vi "Hud_Blit.vi"(0 "Picture":u8[][](array[numeric]), 5 "Sprites":cluster{"Pix":u8[][], "Mask":u8[][]}[](array[cluster]), 7 "State":T1={"Tick"=0, "Phase"=0, "PhaseTicks"=0, "Level"=1, "Room"=0, "X10"=0, "Y10"=0, "VY10"=0, "Mode"=0, "Facing"=0, "Run"=0, "Vert"=0, "StandY"=0, "EntryX10"=0, "EntryY10"=0, "EntryMode"=0, "Lives"=4, "Score"=0, "NextLife"=10000, "KeyR"=0, "KeyB"=0, "KeyY"=0, "Torch"=FALSE, "FloorPhase"=0, "Dead"=FALSE, "LevelStart"=FALSE, "Quit"=FALSE, "Sound"=0, "Seed"=12345, "DemoStep"=0, "Tiles"=[], "World"=[], "Enemies"=[], "Highscores"=[], "Name"=[0, 0, 0], "Cursor"=0}, 11 "error in":errorcluster) -> (4 "Picture out":u8[][](array[numeric]), 15 "error out":errorcluster)   [LabVIEW 2020, in "GH_Render.lvlib"]
doc: "Draws the HUD values into the screen raster (the HUD image itself is already there): lives (at most 7 heads), keys with their number, the torch, level, gold (score) and in the treasure room the seconds left."
uses:
  GH_Render.lvlib
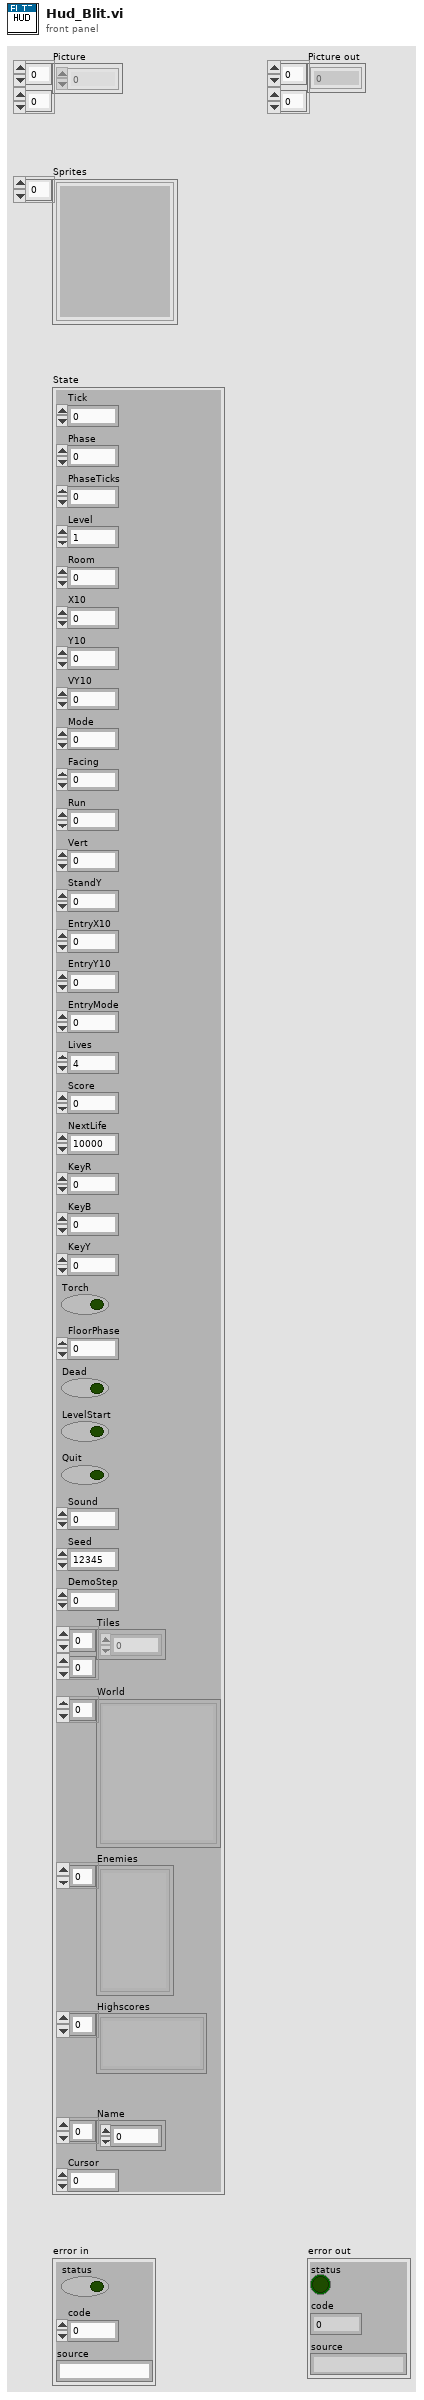
[diagram p1: front panel]
types:
  T1 = cluster{"Tick":u32, "Phase":i32, "PhaseTicks":i32, "Level":i32, "Room":i32, "X10":i32, "Y10":i32, "VY10":i32, "Mode":i32, "Facing":i32, "Run":i32, "Vert":i32, "StandY":i32, "EntryX10":i32, "EntryY10":i32, "EntryMode":i32, "Lives":i32, "Score":i32, "NextLife":i32, "KeyR":i32, "KeyB":i32, "KeyY":i32, "Torch":bool, "FloorPhase":i32, "Dead":bool, "LevelStart":bool, "Quit":bool, "Sound":i32, "Seed":u32, "DemoStep":i32, "Tiles":u8[][], "World":cluster{"ID":string, "Depth":i32, "Column":i32, "Tiles":u8[][]}[], "Enemies":cluster{"Kind":i32, "X10":i32, "Y10":i32, "Dir":i32, "Mode":i32}[], "Highscores":cluster{"Score":i32, "Name":string}[], "Name":i32[], "Cursor":i32}
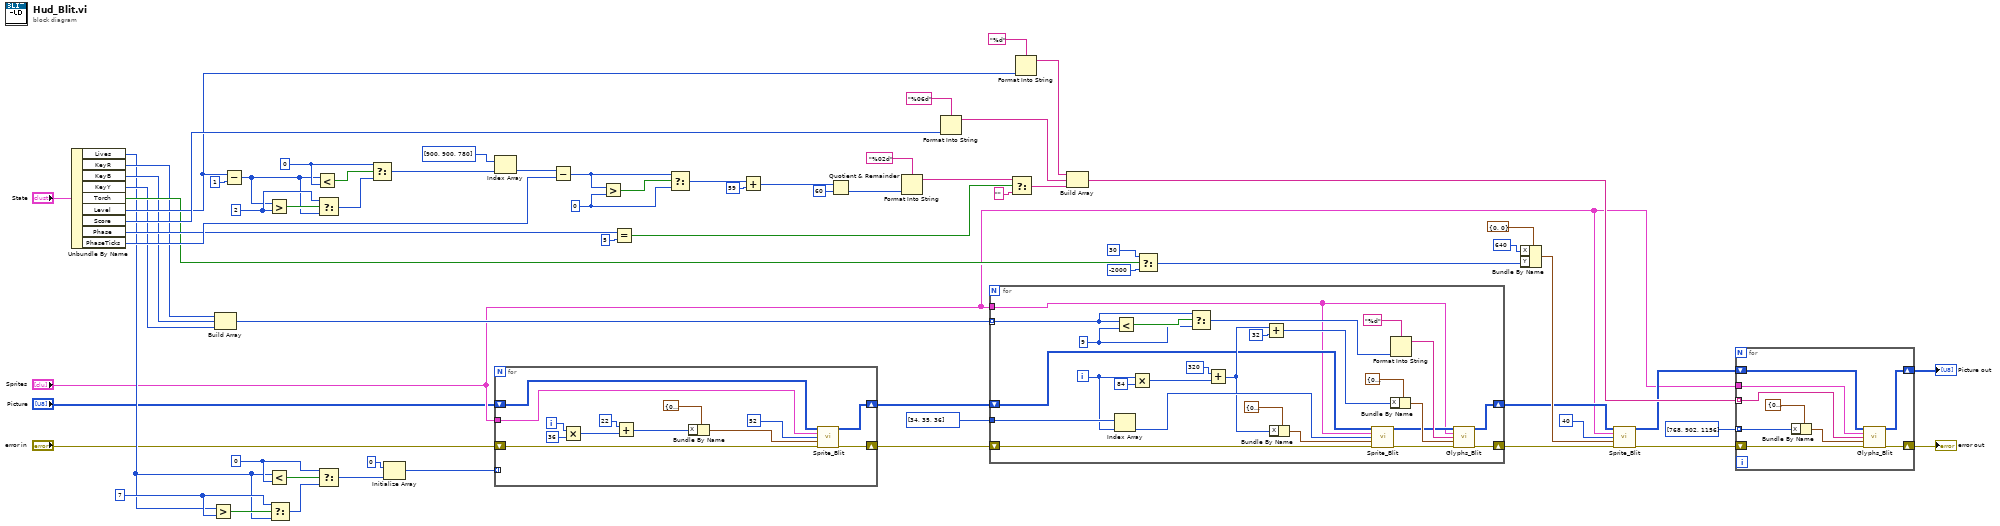
[diagram p0: block diagram]
diagram:
  w48 = 0
  w41 = 2
  w40 = 0
  w15 = 7
  w14 = 0
  n1 = Unbundle By Name("State") -> ("Lives"=w5:i32, "KeyR"=w6:i32, "KeyB"=w7:i32, "KeyY"=w8:i32, "Torch"=w9:bool, "Level"=w10:i32, "Score"=w11:i32, "Phase"=w12:i32, "PhaseTicks"=w13:i32)
  n2 = Greater?(x=w5, y=w15) -> (0:w17:bool)
  n3 = Build Array(w6, w7, w8) -> (w24:i32[])
  n4 = Subtract(x=w10, y=1) -> (x-y=w39:i32)
  n5 = Greater?(x=w39, y=w41) -> (0:w43:bool)
  n6 = Less?(x=w5, y=w14) -> (x < y?=w16:bool)
  n7 = Select(t=w15, s=w17, f=w5) -> (s? t:f=w18:i32)
  n8 = Less?(x=w39, y=w40) -> (x < y?=w42:bool)
  n9 = Select(t=w41, s=w43, f=w39) -> (s? t:f=w44:i32)
  n10 = Select(t=w14, s=w16, f=w18) -> (s? t:f=w19:i32)
  n11 = Select(t=w40, s=w42, f=w44) -> (s? t:f=w45:i32)
  n12 = Initialize Array(0, w19) -> (w21:i32[])
  n13 = Index Array(array=i32[] [900, 900, 780] ("Treasure time"), index=w45) -> (element=w46:i32)
  n14 = for {
    tunnel: "Sprites" -> [w70]
    shift-right: [w72] -> w22
    shift-left: "Picture" -> [w71]
    shift-right: [w74] -> w23
    shift-left: "error in" -> [w73]
    tunnel: w21 -> [_] mode=indexing
    i -> [w69]
    n15 = Multiply(x=w69, y=36) -> (x*y=w79:i32)
    n16 = Add(x=22, y=w79) -> (x+y=w80:i32)
    n17 = Bundle By Name(cluster=cluster{"X":i32, "Y":i32} {"X"=0, "Y"=30}, "X"=w80) -> (w81:cluster{"X":i32, "Y":i32})
    n18 = call "Sprite_Blit.vi"("Picture"=w71, "Sprites"=w70, "Index"=52, "Position"=w81, "error in"=w73) -> ("Picture out"=w72:u8[][], "error out"=w74:errorcluster)  [unwired: 9 in]
  }
  n19 = Subtract(x=w46, y=w13) -> (x-y=w47:i32)
  n20 = Greater?(x=w47, y=w48) -> (0:w49:bool)
  n21 = Equal?(x=w12, y=5) -> (x = y?=w56:bool)
  n22 = Select(t=w47, s=w49, f=w48) -> (s? t:f=w50:i32)
  n23 = Add(x=w50, y=59) -> (x+y=w52:i32)
  n24 = Quotient & Remainder(x=w52, y=60) -> (floor(x/y)=w54:i32)  [unwired: 1 out]
  n25 = Format Into String(format string="%02d", w54) -> (resulting string=w58:string)  [unwired: 2 in, 1 out]
  n26 = Format Into String(format string="%06d", w11) -> (resulting string=w64:string)  [unwired: 2 in, 1 out]
  n27 = for {
    tunnel: i32[] [34, 35, 36] ("Key sprites") -> [w84]
    tunnel: "Sprites" -> [w85]
    shift-right: [w87] -> w26
    shift-left: w22 -> [w86]
    shift-right: [w89] -> w27
    shift-left: w23 -> [w88]
    tunnel: w24 -> [w83] mode=indexing
    i -> [w82]
    w99 = 9
    n28 = Index Array(array=w84, index=w82) -> (element=w94:i32)
    n29 = Less?(x=w83, y=w99) -> (x < y?=w100:bool)
    n30 = Multiply(x=w82, y=84) -> (x*y=w92:i32)
    n31 = Select(t=w83, s=w100, f=w99) -> (s? t:f=w101:i32)
    n32 = Add(x=320, y=w92) -> (x+y=w93:i32)
    n33 = Add(x=w93, y=32) -> (x+y=w106:i32)
    n34 = Bundle By Name(cluster=cluster{"X":i32, "Y":i32} {"X"=0, "Y"=30}, "X"=w93) -> (w96:cluster{"X":i32, "Y":i32})
    n35 = call "Sprite_Blit.vi"("Picture"=w86, "Sprites"=w85, "Index"=w94, "Position"=w96, "error in"=w88) -> ("Picture out"=w97:u8[][], "error out"=w98:errorcluster)  [unwired: 9 in]
    n36 = Format Into String(format string="%d", w101) -> (resulting string=w103:string)  [unwired: 2 in, 1 out]
    n37 = Bundle By Name(cluster=cluster{"X":i32, "Y":i32} {"X"=0, "Y"=30}, "X"=w106) -> (w107:cluster{"X":i32, "Y":i32})
    n38 = call "Glyphs_Blit.vi"("Picture"=w97, "Sprites"=w85, "Text"=w103, "Position"=w107, "error in"=w98) -> ("Picture out"=w87:u8[][], "error out"=w89:errorcluster)  [unwired: 9 in]
  }
  n39 = Select(t=w58, s=w56, f="") -> (s? t:f=w60:string)
  n40 = Format Into String(format string="%d", w10) -> (resulting string=w62:string)  [unwired: 2 in, 1 out]
  n41 = Build Array(w62, w64, w60) -> (w65:string[])
  n42 = Select(t=30, s=w9, f=-2000) -> (s? t:f=w32:i32)
  n43 = Bundle By Name(cluster=cluster{"X":i32, "Y":i32} {"X"=0, "Y"=0}, "X"=640, "Y"=w32) -> (w34:cluster{"X":i32, "Y":i32})
  n44 = call "Sprite_Blit.vi"("Picture"=w26, "Sprites"="Sprites", "Index"=40, "Position"=w34, "error in"=w27) -> ("Picture out"=w35:u8[][], "error out"=w36:errorcluster)  [unwired: 9 in]
  n45 = for {
    tunnel: i32[] [768, 902, 1156] ("Text X") -> [w109] mode=indexing
    tunnel: "Sprites" -> [w110]
    shift-right: [w112] -> w67
    shift-left: w35 -> [w111]
    shift-right: [w114] -> w68
    shift-left: w36 -> [w113]
    tunnel: w65 -> [w108] mode=indexing
    n46 = Bundle By Name(cluster=cluster{"X":i32, "Y":i32} {"X"=0, "Y"=30}, "X"=w109) -> (w116:cluster{"X":i32, "Y":i32})
    n47 = call "Glyphs_Blit.vi"("Picture"=w111, "Sprites"=w110, "Text"=w108, "Position"=w116, "error in"=w113) -> ("Picture out"=w112:u8[][], "error out"=w114:errorcluster)  [unwired: 9 in]
  }
  "Picture out" <- w67
  "error out" <- w68
